vi "Scale List Menu Action.vi"(8 "error in (no error)":errorcluster, 9 "Scale Index":i32, 10 "ItemTag":string, 11 "Data Viewer in":refnum<class "Data Viewer.lvclass">) -> (0 "error out":errorcluster, 3 "Data Viewer out":refnum<class "Data Viewer.lvclass">)   [LabVIEW 2020, in "Data Viewer.lvlib" / "Data Viewer.lvclass"]
uses:
  Data Viewer.lvclass
  Data Viewer.lvclass/Data Viewer.ctl
  Scale Setting--cluster.ctl
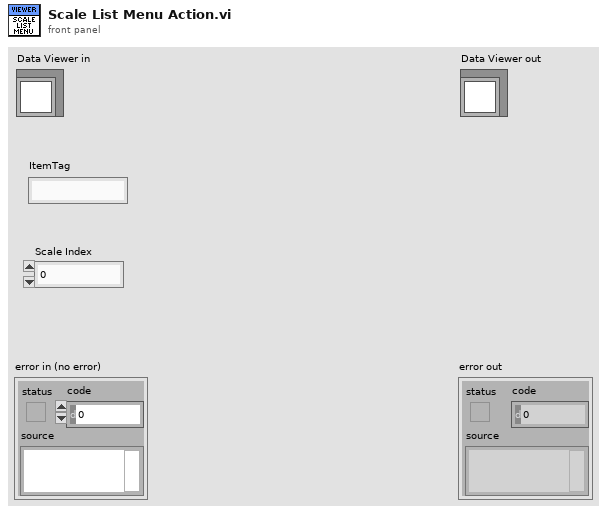
[diagram p1: front panel]
types:
  T1 = typedef "Data Viewer.lvlib/Data Viewer.lvclass/Scale Setting--cluster.ctl" = cluster{"Name":string, "Unit":string, "Color":u32, "Auto Scale":bool, "Scale Min":dbl, "Scale Max":dbl, "Scale Interval":dbl, "Show Gird":bool, "Log":bool}
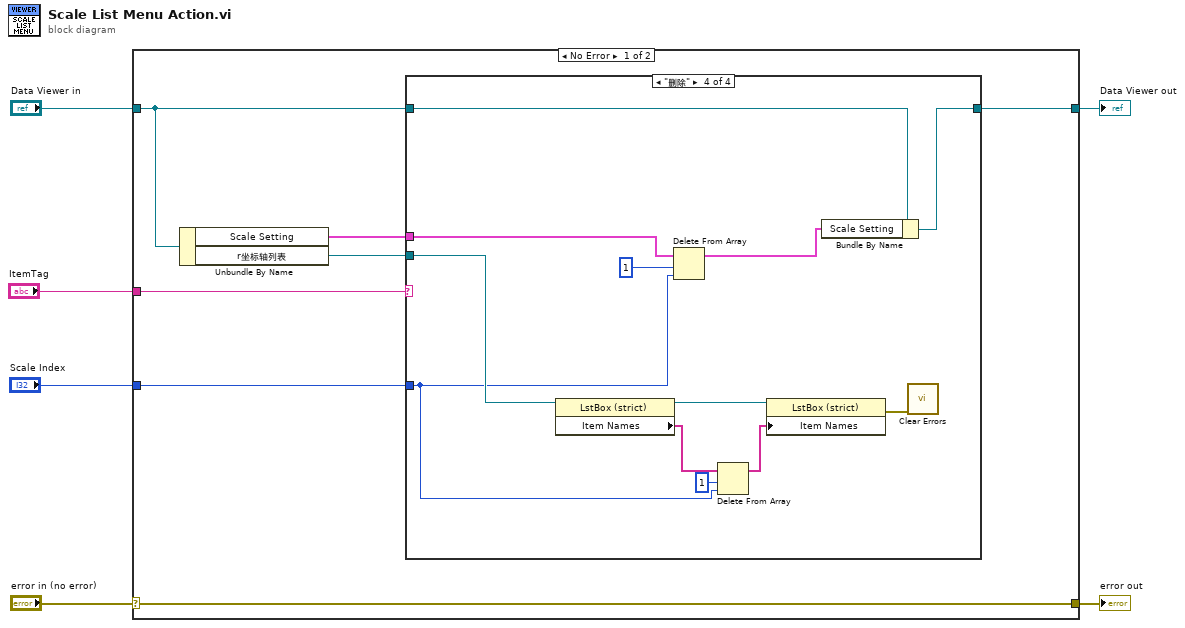
[diagram p0: block diagram]
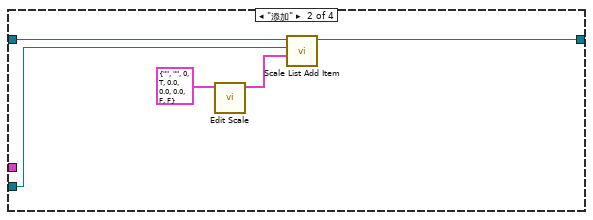
[diagram p3: hidden frame]
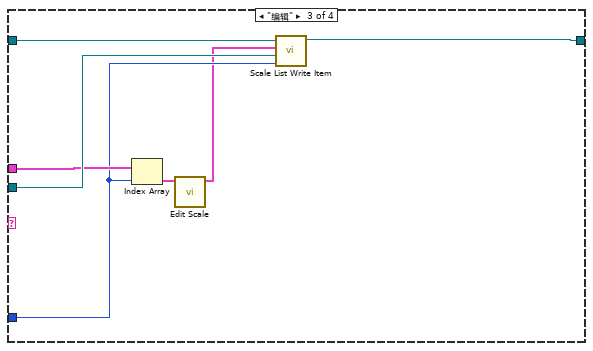
[diagram p4: hidden frame]
diagram:
  n1 = case shown="No Error" "error in (no error)" {
    selector: "error in (no error)" -> [w13 w40]
    tunnel: [w13 w40] -> w5
    tunnel: [w8 w39] -> w3
    tunnel: "Data Viewer in" -> [w9 w39]
    tunnel: "ItemTag" -> [w12 _]
    tunnel: "Scale Index" -> [w11 _]
    frame No Error {
      n2 = Unbundle By Name(w9) -> ("Scale Setting"=w10:T1[], "r坐标轴列表"=w7:refnum<vi>)
      n3 = case shown="\"删除\"" w12 {
        tunnel: w11 -> [_ _ w22 w28]
        tunnel: w10 -> [_ _ w23 w31]
        tunnel: w9 -> [w14 w18 w26 w34]
        tunnel: [w14 w17 w25 w30] -> w8
        tunnel: w7 -> [_ w16 w24 w33]
        frame "False", Default {
        }
        frame "添加" {
          n4 = call "Edit Scale.vi"("Sacle Setting In"=T1 {"Name"="", "Unit"="", "Color"=0, "Auto Scale"=TRUE, "Scale Min"=0.0, "Scale Max"=0.0, "Scale Interval"=0.0, "Show Gird"=FALSE, "Log"=FALSE}) -> ("Sacle Setting Out"=w15:T1)  [unwired: 10 in]
          n5 = call "Scale List Add Item.vi"("Sacle Setting Out"=w15, "r坐标轴列表"=w16, "Data Viewer in"=w18) -> ("Data Viewer out"=w17:refnum<class "Data Viewer.lvclass">)  [unwired: 8 in]
        }
        frame "编辑" {
          n6 = Index Array(array=w23, index=w22) -> (element=w21:T1)
          n7 = call "Edit Scale.vi"("Sacle Setting In"=w21) -> ("Sacle Setting Out"=w20:T1)  [unwired: 10 in]
          n8 = call "Scale List Write Item.vi"("Scale Index"=w22, "r坐标轴列表"=w24, "Sacle Setting"=w20, "Data Viewer in"=w26) -> ("Data Viewer out"=w25:refnum<class "Data Viewer.lvclass">)  [unwired: 7 in]
        }
        frame "删除" {
          n9 = property class="LstBox (strict)"(reference=w33) -> (reference out=w35:refnum<vi>, "Item Names"=w38:string[])  [unwired: 1 in, 1 out]
          n10 = Delete From Array(array=w31, length=1, index=w28) -> (array with subset deleted=w29:T1[])  [unwired: 1 out]
          n11 = Delete From Array(array=w38, length=1, index=w28) -> (array with subset deleted=w36:string[])  [unwired: 1 out]
          n12 = property class="LstBox (strict)"(reference=w35, "Item Names"=w36) -> (error out=w27:errorcluster)  [unwired: 1 in, 1 out]
          n13 = Bundle By Name(cluster=w34, "Scale Setting"=w29) -> (w30:refnum<class "Data Viewer.lvclass">)
          n14 = call <vilib>:"Clear Errors.vi"("error in (no error)"=w27) -> ()  [unwired: 5 in, 2 out]
        }
      }
    }
    frame Error {
    }
  }
  "error out" <- w5
  "Data Viewer out" <- w3
